vi "FilterArray.vi"(1 "Items to Filter":string[](array[string]), 2 "Items to Exclude":string[](array[string])) -> (0 "Filtered Array":string[](array[string]))   [LabVIEW 2023]
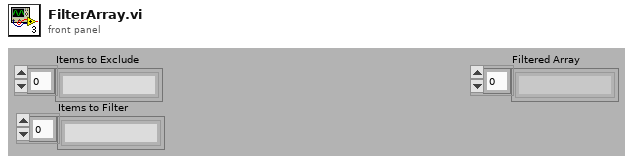
[diagram p1: front panel]
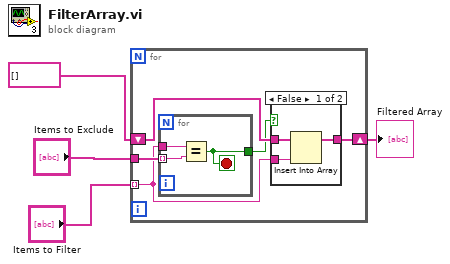
[diagram p0: block diagram]
diagram:
  n1 = for {
    tunnel: "Items to Filter" -> [w5] mode=indexing
    tunnel: "Items to Exclude" -> [w9]
    shift-right: [w7] -> w1
    shift-left: string[] [] -> [w8]
    n2 = for {
      tunnel: w9 -> [w16] mode=indexing
      tunnel: w5 -> [w14]
      tunnel: [w15] -> w6
      stop <- w15 stop-if-true
      n3 = Equal?(x=w14, y=w16) -> (x = y?=w15:bool)
    }
    n4 = case shown="False" w6 {
      tunnel: w8 -> [w12 w13]
      tunnel: [w11 w13] -> w7
      tunnel: w5 -> [w10 _]
      frame False {
        n5 = Insert Into Array(array=w12, new element=w10) -> (w11:string[])  [unwired: 1 in]
      }
      frame True {
      }
    }
  }
  "Filtered Array" <- w1
